vi "Random Chance.vi"(11 "probability":dbl) -> (3 "happened?":bool)   [LabVIEW 2020, in "Full Featured MCP Server.lvlib"]
doc: "Rolls the dice: happened? is TRUE with the given probability (0 = never, 1 = always)."
uses:
  Full Featured MCP Server.lvlib
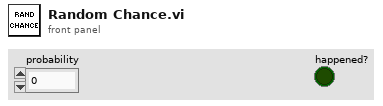
[diagram p1: front panel]
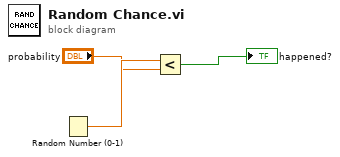
[diagram p0: block diagram]
diagram:
  n1 = Random Number (0-1)() -> (number: 0 to 1=w2:dbl)
  n2 = Less?(x=w2, y="probability") -> (x < y?=→"happened?":bool)
